vi "Finalize Hardware.vi"(6 "force (F)":bool, 8 "error in":errorcluster, 11 "board identifier":u8) -> (0 "error out":errorcluster)   [LabVIEW 2020, in "AIM ARINC 429 Hardware API.lvlib"]
uses:
  AIM ARINC 429 Hardware API.lvlib
  <instrlib>/AIM GmbH/_ARINC-429/Controls/HwManager_action.ctl
  <instrlib>/AIM GmbH/_ARINC-429/AIM429LV.lvlib
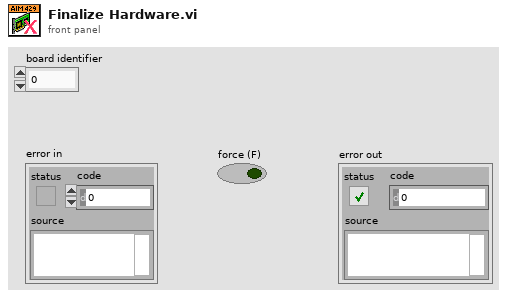
[diagram p1: front panel]
types:
  T1 = typedef "AIM429LV.lvlib/HwManager_action.ctl" = enum16{"Get Resource", "Remove Instance", "Add Resource", "Clear All", "Remove Resource"}
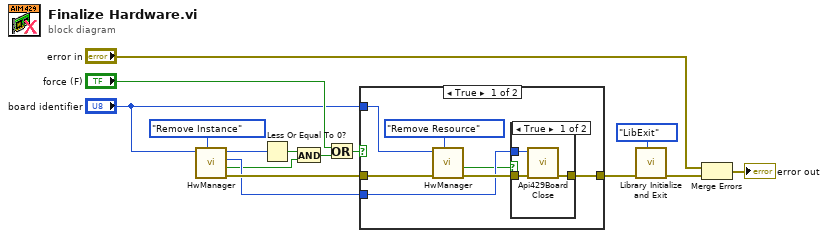
[diagram p0: block diagram]
diagram:
  n1 = call <instrlib>:"HwManager.vi"("Action (Get)"=HwManager_action."Remove Instance", "board id"="board identifier") -> ("error out"=w12:errorcluster, "found"=w4:bool, "module handle out"=w5:u8, "# of board instances"=w13:i32)  [unwired: 6 in]
  n2 = Less Or Equal To 0?(x=w13) -> (x <= 0?=w7:bool)
  n3 = And(x=w7, y=w4) -> (x .and. y?=w6:bool)
  n4 = Or(x="force (F)", y=w6) -> (x .or. y?=w8:bool)
  n5 = case shown="True" w8 {
    tunnel: w12 -> [w22 w27]
    tunnel: "board identifier" -> [w20 _]
    tunnel: [w18 w27] -> w3
    tunnel: w5 -> [w17 _]
    frame True {
      n6 = call <instrlib>:"HwManager.vi"("Action (Get)"=HwManager_action."Remove Resource", "error in (no error)"=w22, "board id"=w20) -> ("error out"=w19:errorcluster, "found"=w16:bool)  [unwired: 5 in, 2 out]
      n7 = case shown="True" w16 {
        tunnel: w19 -> [w24 w26]
        tunnel: [w25 w26] -> w18
        tunnel: w17 -> [w23 _]
        frame True {
          n8 = call <instrlib>:"Api429Board Close.vi"("error in (no error)"=w24, "board_handle"=w23) -> ("error out"=w25:errorcluster)  [unwired: 9 in]
        }
        frame False {
        }
      }
    }
    frame False {
    }
  }
  n9 = call "Library Initialize and Exit.vi"("action"=enum16{"LibInit", "LibExit"}."LibExit", "error in"=w3) -> ("error out"=w2:errorcluster)  [unwired: 7 in, 2 out]
  n10 = Merge Errors("error in", w2) -> (→"error out":errorcluster)
